vi "Sort (multiple).vi"(8 "error in (no error)":errorcluster, 9 "Use Sort Pointers (F)":bool, 10 "Sort Pointers":i32[](array[numeric]), 11 "XY-data":cluster{"X-array":dbl[], "Y-array":dbl[]}[](array[cluster]) {"Y-array" format="%.2p"; "X-array" format="%.2p"}) -> (0 "error out":errorcluster, 2 "Sorted Pointers":i32[](array[numeric]), 3 "Sorted XY-data out":cluster{"X-array":dbl[], "Y-array":dbl[]}[](array[cluster]) {"Y-array" format="%.2p"; "X-array" format="%.2p"})   [LabVIEW 2019, in "xy_utilities.lvlib"]
doc: "Sorts the input <b>XY-data</b> according to its x array.\n\nIf <b>Use Sort Pointers</b> = <b>True</b> then sort according to <b>Sort Pointers</b>.\n\nWire data to the data input to determine the polymorphic instance to use or manually select the instance."
uses:
  xy_utilities.lvlib
  <userlib>/_OpenG.lib/array/array.llb/Sort Array__ogtk.vi
  <userlib>/_OpenG.lib/array/array.llb/Sort 1D Array (DBL)__ogtk.vi
  <userlib>/_OpenG.lib/array/array.llb/Reorder Array2__ogtk.vi
  <userlib>/_OpenG.lib/array/array.llb/Reorder 1D Array2 (DBL)__ogtk.vi
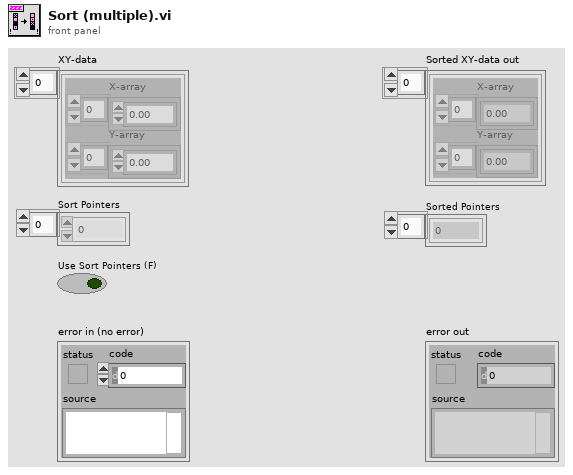
[diagram p1: front panel]
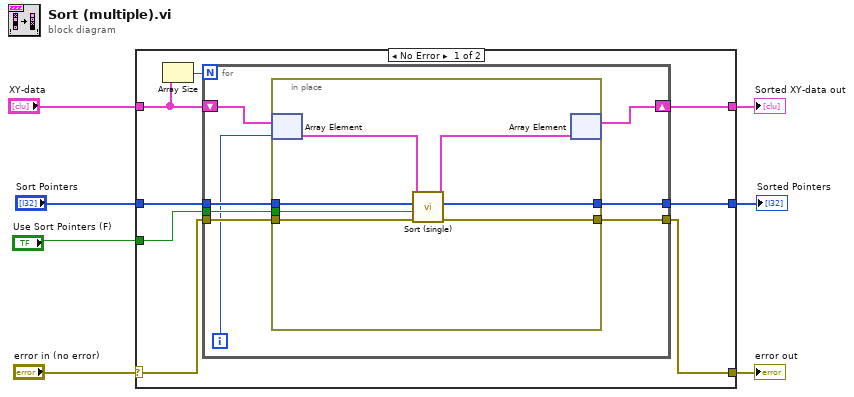
[diagram p0: block diagram]
diagram:
  n1 = case shown="No Error" "error in (no error)" {
    selector: "error in (no error)" -> [w13 w33]
    tunnel: [w14 w33] -> w6
    tunnel: "XY-data" -> [w8 w32]
    tunnel: [w15 w32] -> w4
    tunnel: [w12 w31] -> w1
    tunnel: "Use Sort Pointers (F)" -> [w11 _]
    tunnel: "Sort Pointers" -> [w10 w31]
    frame No Error {
      n2 = Array Size(array=w8) -> (size(s)=w9:i32)
      n3 = for {
        N: w9 -> [_]
        tunnel: [w21] -> w12
        tunnel: w11 -> [w20]
        tunnel: w10 -> [w19]
        tunnel: w13 -> [w22]
        tunnel: [w23] -> w14
        shift-right: [w17] -> w15
        shift-left: w8 -> [w18]
        i -> [w16]
        n4 = in-place {
          in-place-border: [w30] -> w23
          in-place-border: w22 -> [w29]
          in-place-border: [w28] -> w21
          in-place-border: w20 -> [w27]
          in-place-border: w19 -> [w26]
          n5 = in-place-array #1(w18, w16) -> (w25:cluster{"X-array":dbl[], "Y-array":dbl[]})
          n6 = call "Sort (single).vi"("error in (no error)"=w29, "Use Sort Pointers (F)"=w27, "Sort Pointers"=w26, "XY-data"=w25) -> ("error out"=w30:errorcluster, "Sorted Pointers"=w28:i32[], "Sorted XY-data out"=w24:cluster{"X-array":dbl[], "Y-array":dbl[]})  [unwired: 5 in]
          n7 = in-place-array #1(w24) -> (w17:cluster{"X-array":dbl[], "Y-array":dbl[]}[])  [unwired: 1 out]
        }
      }
    }
    frame Error {
    }
  }
  "error out" <- w6
  "Sorted XY-data out" <- w4
  "Sorted Pointers" <- w1
